vi "Tree_FocusTag_Tests.vi"(11 "error in":errorcluster) -> (15 "error out":errorcluster)   [LabVIEW 2016, in "DronaTest.lvlib"]
uses:
  DronaTest.lvlib
  APIs/Stimulus/ControlValue/SetValueAuto.vi
  APIs/Stimulus/ControlValue/Controls/Tree/SetValueByItemTag.vi
  APIs/Assert/AssertControlValue/Controls/Tree/AssertValueByFocusTag.vi
  <vilib>/addons/_JKI Toolkits/Caraya/classes/Assert/Assert Equal Value_Variant.vi
  <vilib>/addons/_JKI Toolkits/Caraya/classes/Assert/Assert Error.vi
  <vilib>/addons/_JKI Toolkits/Caraya/classes/Test/Test.lvclass
  Drona.lvlib
  <vilib>/SLL Toolkit/SLL Debug/SLL Debug.lvlib
  <vilib>/addons/_JKI Toolkits/Caraya/classes/Assert/Assert.lvclass
  APIs/Stimulus/ControlValue/Controls/Tree/StimulusTree.lvlib
  APIs/Assert/AssertControlValue/Controls/Tree/AssertTree.lvlib
  APIs/Stimulus/ControlValue/ControlValue.lvlib
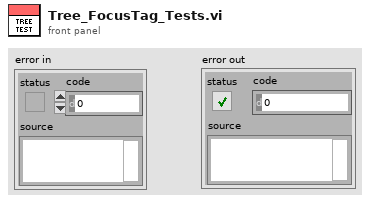
[diagram p1: front panel]
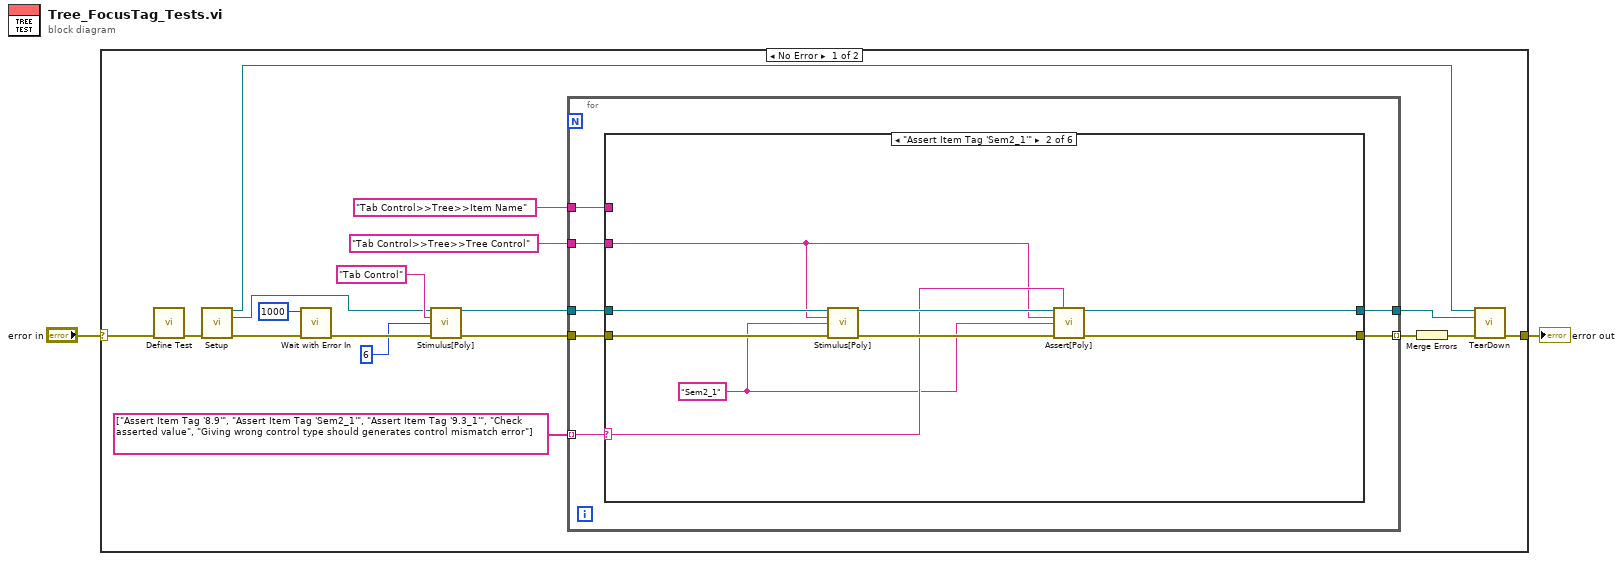
[diagram p0: block diagram]
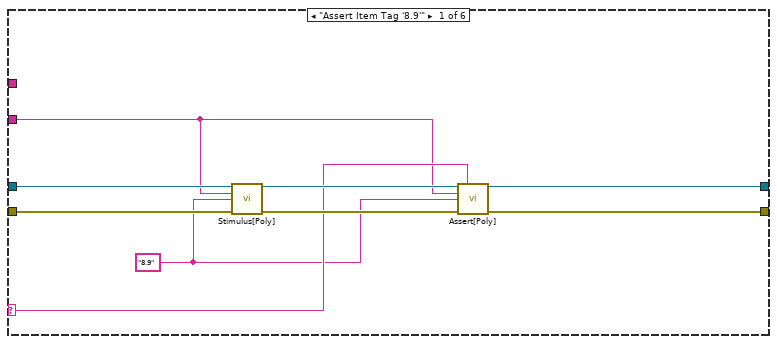
[diagram p2: hidden frame]
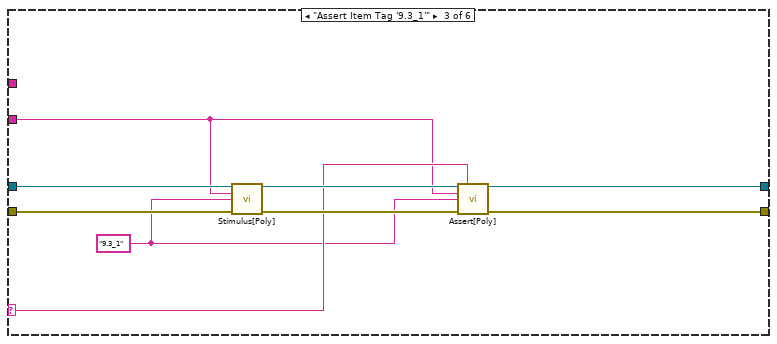
[diagram p3: hidden frame]
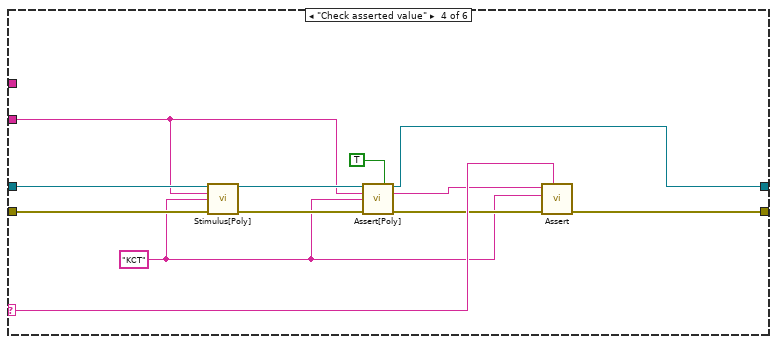
[diagram p4: hidden frame]
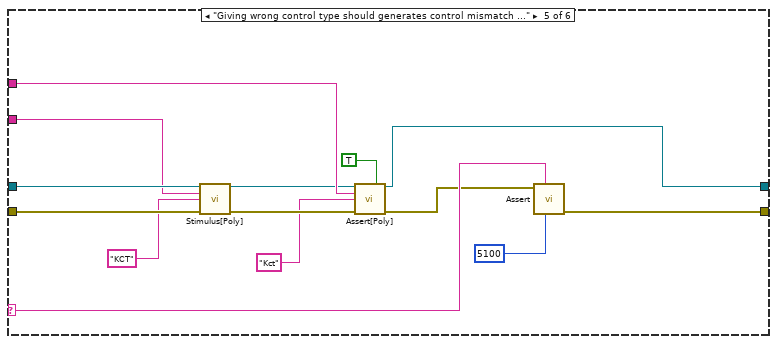
[diagram p5: hidden frame]
diagram:
  n1 = case shown="No Error" "error in" {
    selector: "error in" -> [w20 w83]
    tunnel: [w3 w83] -> w1
    frame No Error {
      n2 = call <vilib>:"Define Test.vi"("error in (no error)"=w20) -> ("error out"=w9:errorcluster)  [unwired: 9 in, 1 out]
      n3 = call "Setup.vi"("error in"=w9) -> ("Application Ref"=w4:refnum<vi>, "VI out"=w8:refnum<vi>, "error out"=w7:errorcluster)  [unwired: 12 in]
      n4 = call <vilib>:"Wait with Error In.vi"("error in (no error)"=w7, "milliseconds to wait"=u32 1000) -> ("error out"=w18:errorcluster)  [unwired: 9 in]
      n5 = call-poly "Stimulus[Poly].vi"("VI Reference In"=w8, "Control Path"="Tab Control", "Value (Signaling)"=6, "error in"=w18) -> ("VI Reference Out"=w14:refnum<vi>, "error out"=w17:errorcluster)  [unwired: 10 in]
      n6 = for {
        tunnel: w14 -> [w26]
        tunnel: "Tab Control>>Tree>>Tree Control" ("Control Path") -> [w25]
        tunnel: "Tab Control>>Tree>>Item Name" ("Control Path") -> [w24]
        tunnel: string[] ["Assert Item Tag '8.9'", "Assert Item Tag 'Sem2_1'", "Assert Item Tag '9.3_1'", "Check asserted value", "Giving wrong control type should generates control mismatch error"] -> [w22] mode=indexing
        tunnel: [w21] -> w5
        tunnel: w17 -> [w27]
        tunnel: [w23] -> w10 mode=indexing
        n7 = case shown="\"Assert Item Tag 'Sem2_1'\"" w22 {
          selector: w22 -> [w30 w39 w48 w63 w77 _]
          tunnel: w27 -> [w36 w45 w54 w66 w80 w82]
          tunnel: w26 -> [w35 w44 w53 w65 w79 w81]
          tunnel: w25 -> [w28 w37 w47 w59 w75 _]
          tunnel: w24 -> [_ _ _ _ w73 _]
          tunnel: [w32 w41 w50 w64 w78 w82] -> w23
          tunnel: [w31 w40 w49 w60 w70 w81] -> w21
          frame "Assert Item Tag '8.9'" {
            w29 = "8.9" ("Item Name")
            n8 = call-poly "Stimulus[Poly].vi"("VI Reference In"=w35, "Control Path"=w28, "Item Tag"=w29, "Error In"=w36) -> ("VI Reference Out"=w33:refnum<vi>, "Error Out"=w34:errorcluster)  [unwired: 10 in]
            n9 = call-poly "Assert[Poly].vi"("VI Reference In"=w33, "Test Label"=w30, "Control Path"=w28, "Focus Item Tag"=w29, "Error In"=w34) -> ("VI Reference Out"=w31:refnum<vi>, "Error Out"=w32:errorcluster)  [unwired: 8 in, 1 out]
          }
          frame "Assert Item Tag 'Sem2_1'" {
            w38 = "Sem2_1" ("Item Name")
            n10 = call-poly "Stimulus[Poly].vi"("VI Reference In"=w44, "Control Path"=w37, "Item Tag"=w38, "Error In"=w45) -> ("VI Reference Out"=w42:refnum<vi>, "Error Out"=w43:errorcluster)  [unwired: 10 in]
            n11 = call-poly "Assert[Poly].vi"("VI Reference In"=w42, "Test Label"=w39, "Control Path"=w37, "Focus Item Tag"=w38, "Error In"=w43) -> ("VI Reference Out"=w40:refnum<vi>, "Error Out"=w41:errorcluster)  [unwired: 8 in, 1 out]
          }
          frame "Assert Item Tag '9.3_1'" {
            w46 = "9.3_1" ("Item Name")
            n12 = call-poly "Stimulus[Poly].vi"("VI Reference In"=w53, "Control Path"=w47, "Item Tag"=w46, "Error In"=w54) -> ("VI Reference Out"=w51:refnum<vi>, "Error Out"=w52:errorcluster)  [unwired: 10 in]
            n13 = call-poly "Assert[Poly].vi"("VI Reference In"=w51, "Test Label"=w48, "Control Path"=w47, "Focus Item Tag"=w46, "Error In"=w52) -> ("VI Reference Out"=w49:refnum<vi>, "Error Out"=w50:errorcluster)  [unwired: 8 in, 1 out]
          }
          frame "Check asserted value" {
            w56 = "KCT" ("Item Name")
            n14 = call-poly "Stimulus[Poly].vi"("VI Reference In"=w65, "Control Path"=w59, "Item Tag"=w56, "Error In"=w66) -> ("VI Reference Out"=w61:refnum<vi>, "Error Out"=w62:errorcluster)  [unwired: 10 in]
            n15 = call-poly "Assert[Poly].vi"("VI Reference In"=w61, "Assert Only? (F)"=TRUE, "Control Path"=w59, "Focus Item Tag"=w56, "Error In"=w62) -> ("VI Reference Out"=w60:refnum<vi>, "Asserted Value"=w57:string, "Error Out"=w58:errorcluster)  [unwired: 8 in]
            n16 = call-poly <vilib>:"Assert.vi"("Label"=w63, "error in (no error)"=w58, "Y"=w56, "X"=w57) -> ("error out"=w64:errorcluster)  [unwired: 6 in, 1 out]
          }
          frame "Giving wrong control type should generates control mismatch error" {
            n17 = call-poly "Stimulus[Poly].vi"("VI Reference In"=w79, "Control Path"=w75, "Item Tag"="KCT" ("Item Name"), "Error In"=w80) -> ("VI Reference Out"=w71:refnum<vi>, "Error Out"=w74:errorcluster)  [unwired: 10 in]
            n18 = call-poly "Assert[Poly].vi"("VI Reference In"=w71, "Assert Only? (F)"=TRUE, "Control Path"=w73, "Focus Item Tag"="Kct" ("Item Name"), "Error In"=w74) -> ("VI Reference Out"=w70:refnum<vi>, "Error Out"=w69:errorcluster)  [unwired: 8 in, 1 out]
            n19 = call-poly <vilib>:"Assert.vi"("error code (1)"=5100, "Label"=w77, "Error?"=w69) -> ("error out"=w78:errorcluster)  [unwired: 7 in, 1 out]
          }
          frame Default {
          }
        }
      }
      n20 = Merge Errors(w10) -> (w6:errorcluster)
      n21 = call "TearDown.vi"("Application Ref"=w4, "VI in"=w5, "error in (no error)"=w6) -> ("error out"=w3:errorcluster)  [unwired: 12 in]
    }
    frame Error {
    }
  }
  "error out" <- w1
